vi "Delete Filtered Files In Directory.vi"(1 "Error in":errorcluster, 2 "Path":path, 3 "Files to Exclude":string[](array[string]), 4 "Folders to Exclude":string[](array[string])) -> (0 "Error out":errorcluster)   [LabVIEW 2023]
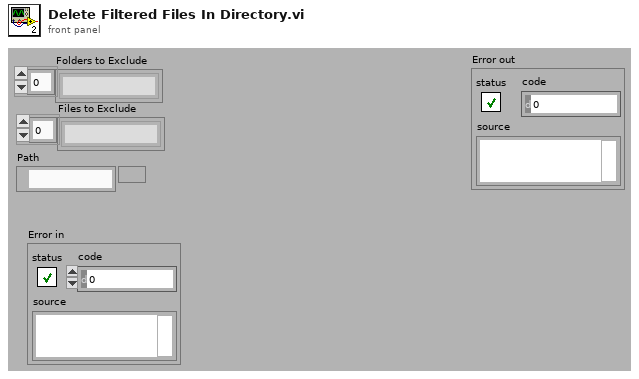
[diagram p1: front panel]
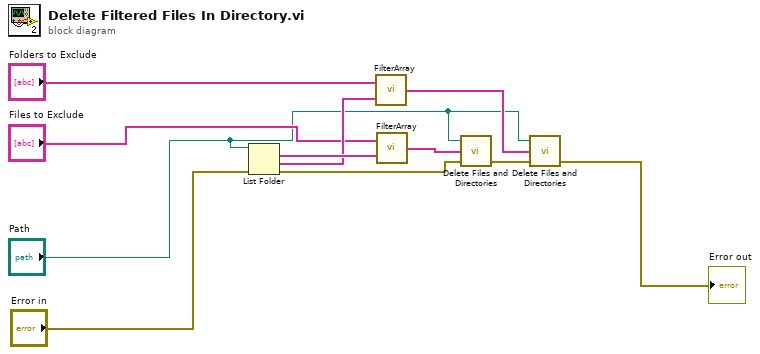
[diagram p0: block diagram]
diagram:
  n1 = List Folder(path="Path", error in="Error in") -> (filenames=w11:string[], folder names=w10:string[], error out=w8:errorcluster)  [unwired: 2 in, 1 out]
  n2 = call <resource>:"FilterArray.vi"("Items to Filter"=w10, "Items to Exclude"="Folders to Exclude") -> ("Filtered Array"=w7:string[])
  n3 = call <resource>:"FilterArray.vi"("Items to Filter"=w11, "Items to Exclude"="Files to Exclude") -> ("Filtered Array"=w9:string[])
  n4 = call <resource>:"Delete Files and Directories.vi"("error in"=w8, "Items to Delete"=w9, "Base path"="Path") -> ("error out"=w6:errorcluster)  [unwired: 2 in]
  n5 = call <resource>:"Delete Files and Directories.vi"("error in"=w6, "Items to Delete"=w7, "Base path"="Path") -> ("error out"=→"Error out":errorcluster)  [unwired: 2 in]
